vi "Delete State.vi"(7 "Delete Callers? (F: Only Delete Case Structure Frame)":bool, 8 "error in (no error)":errorcluster, 9 "State Name":string, 10 "Category (Optional)":string, 11 "JKI SM in":refnum<class "JKI SM.lvclass">) -> (0 "error out":errorcluster, 3 "JKI SM out":refnum<class "JKI SM.lvclass">)   [LabVIEW 2020, in "JKI State Machine API.lvlib" / "JKI SM.lvclass"]
uses:
  JKI SM.lvclass
  JKI SM.lvclass/JKI SM.ctl
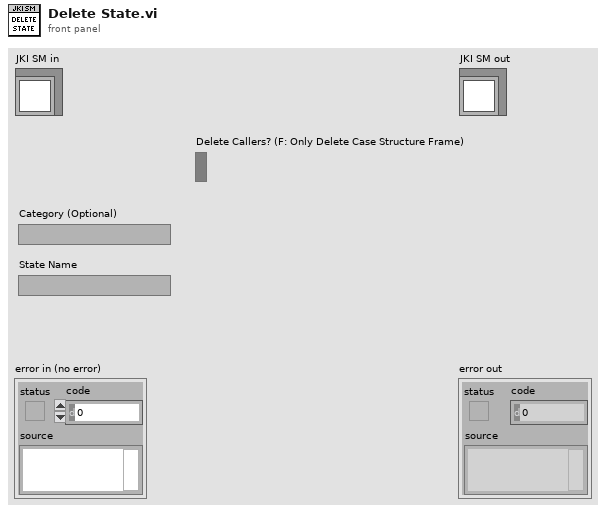
[diagram p1: front panel]
types:
  T1 = cluster{"StringConstant":refnum<vi>, "Structure":string, "Frame Name":string, "State Call":string}[]
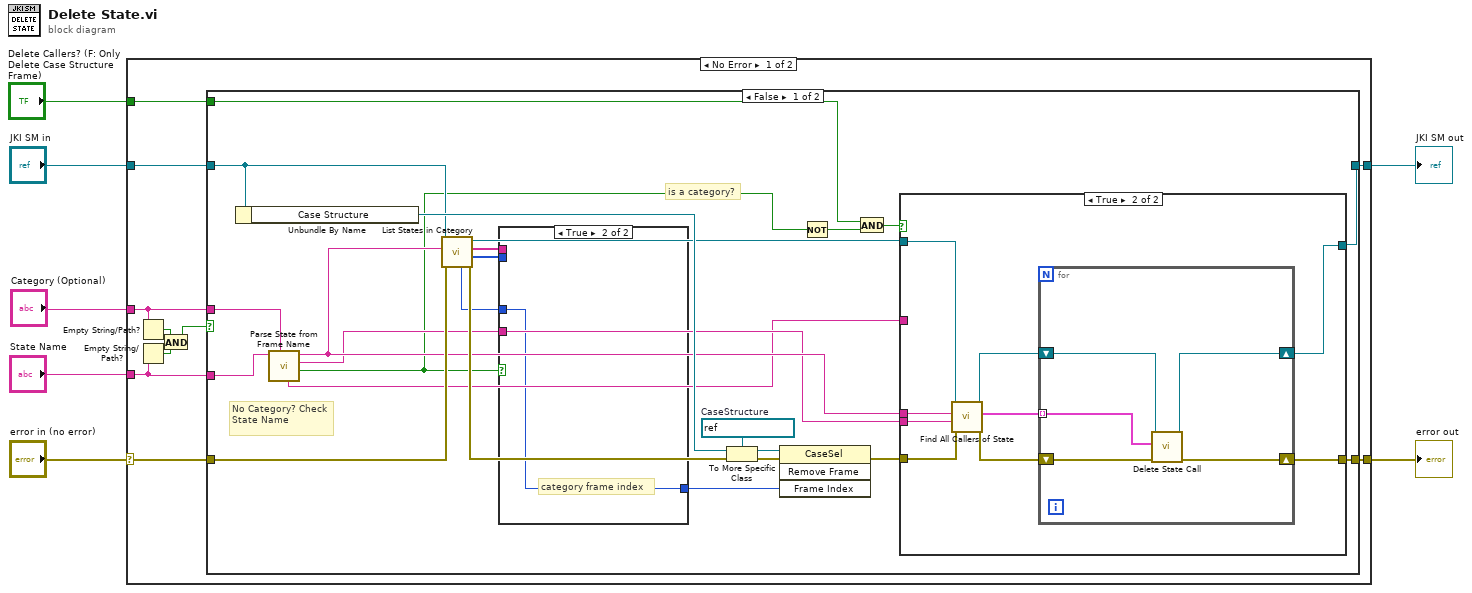
[diagram p0: block diagram]
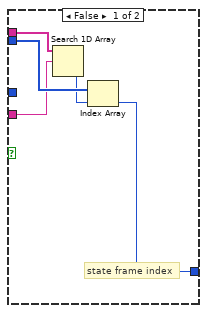
[diagram p2: hidden frame]
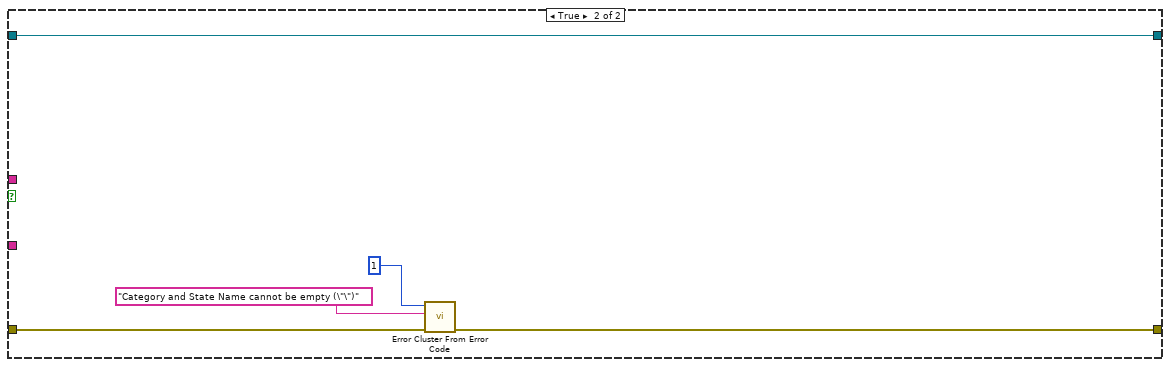
[diagram p4: hidden frame]
diagram:
  n1 = case shown="No Error" "error in (no error)" {
    selector: "error in (no error)" -> [w17 w70]
    tunnel: [w15 w70] -> w6
    tunnel: [w14 w69] -> w4
    tunnel: "JKI SM in" -> [w16 w69]
    tunnel: "State Name" -> [w10 _]
    tunnel: "Category (Optional)" -> [w9 _]
    tunnel: "Delete Callers? (F: Only Delete Case Structure Frame)" -> [w13 _]
    frame No Error {
      n2 = Empty String/Path?(string/path=w9) -> (empty?=w11:bool)
      n3 = Empty String/Path?(string/path=w10) -> (empty?=w12:bool)
      n4 = And(x=w11, y=w12) -> (x .and. y?=w8:bool)
      n5 = case shown="False" w8 {
        tunnel: w17 -> [w34 w67]
        tunnel: w16 -> [w31 w68]
        tunnel: [w29 w66] -> w15
        tunnel: [w28 w68] -> w14
        tunnel: w13 -> [w21 _]
        tunnel: w10 -> [w19 _]
        tunnel: w9 -> [w18 _]
        frame False {
          w39 = refnum<vi> refnum  # CaseStructure
          # "is a category?"
          # "No Category? Check State Name"
          n6 = Unbundle By Name(w31) -> ("Case Structure"=w35:refnum<vi>)
          n7 = call "Parse State from Frame Name.vi"("Category (Optional)"=w18, "Frame or State Name"=w19) -> ("is a Category Frame?"=w22:bool, "State Name"=w26:string, "Category Name"=w27:string, "\"Category: State\" String"=w25:string)  [unwired: 4 in, 2 out]
          n8 = call "List States in Category.vi"("error in (no error)"=w34, "Category"=w27, "JKI SM in"=w31) -> ("error out"=w33:errorcluster, "State Frame Indices"=w37:i32[], "States"=w38:string[], "JKI SM out"=w32:refnum<class "JKI SM.lvclass">, "Category Frame Index"=w24:i32)  [unwired: 4 in]
          n9 = case shown="True" w22 {
            tunnel: w38 -> [w46 _]
            tunnel: w37 -> [w45 _]
            tunnel: [w43 w47] -> w36
            tunnel: w26 -> [w42 _]
            tunnel: w24 -> [_ w47]
            frame False {
              # "state frame index"
              n10 = Search 1D Array(1D array=w46, element=w42) -> (index of element=w44:i32)  [unwired: 1 in]
              n11 = Index Array(array=w45, index=w44) -> (element=w43:i32)
            }
            frame True {
              # "category frame index"
            }
          }
          n12 = To More Specific Class(target class=w39, reference=w35, error in=w33) -> (specific class reference=w40:refnum<vi>, error out=w41:errorcluster)
          n13 = invoke class="CaseSel" method="Remove Frame"(reference=w40, error in=w41, "Frame Index"=w36) -> (error out=w30:errorcluster)  [unwired: 1 in, 3 out]
          n14 = Not(x=w22) -> (.not. x?=w23:bool)
          n15 = And(x=w21, y=w23) -> (x .and. y?=w20:bool)
          n16 = case shown="True" w20 {
            tunnel: w32 -> [w49 w58]
            tunnel: w30 -> [w48 w57]
            tunnel: [w48 w55] -> w29
            tunnel: [w49 w52] -> w28
            tunnel: w27 -> [_ w51]
            tunnel: w26 -> [_ w50]
            tunnel: w25 -> [_ _]
            frame False {
            }
            frame True {
              n17 = call "Find All Callers of State.vi"("error in (no error)"=w57, "State Name"=w50, "Category (Optional)"=w51, "JKI SM in"=w58) -> ("error out"=w54:errorcluster, "Callers"=w56:T1, "JKI SM out"=w53:refnum<class "JKI SM.lvclass">)  [unwired: 5 in]
              n18 = for {
                tunnel: w56 -> [w61] mode=indexing
                shift-right: [w62] -> w55
                shift-left: w54 -> [w63]
                shift-right: [w59] -> w52
                shift-left: w53 -> [w60]
                n19 = call "Delete State Call.vi"("error in (no error)"=w63, "State Call"=w61, "JKI SM in"=w60) -> ("error out"=w62:errorcluster, "JKI SM out"=w59:refnum<class "JKI SM.lvclass">)  [unwired: 7 in]
              }
            }
          }
        }
        frame True {
          n20 = call <vilib>:"Error Cluster From Error Code.vi"("error in (no error)"=w67, "error message (\"\")"="Category and State Name cannot be empty (\"\")" ("error message (\"\")"), "error code (0)"=1) -> ("error out"=w66:errorcluster)  [unwired: 6 in]
        }
      }
    }
    frame Error {
    }
  }
  "error out" <- w6
  "JKI SM out" <- w4
